vi "VIH Project - Container - Item Rules.vi"(6 "cmd (get)":T9(ring), 8 "error in":errorcluster, 9 "Item Rule":T1, 10 "Item Idx (-1)":i32=-1, 11 "Item Path":path) -> (0 "error out":errorcluster, 1 "Item Rule out":T1, 2 "Item Idx out":i32, 3 "Item Path out":path, 5 "Item Paths":path[](array[path]))   [LabVIEW 2014]
doc: "::: VI Helpeks :::\nCopyright (c) 2000-2026 Konstantin Shifershteyn. All rights reserved."
uses:
  _VIH HelpGen.llb/VIH HelpGen Typedef - Cluster - File Rule.ctl
  _VIH HelpGen.llb/VIH HelpGen Typedef - Enum - Default,Enable,Disable.ctl
  _VIH HelpGen.llb/VIH HelpGen Typedef - Cluster - File Rule - Source Paths.ctl
  _VIH HelpGen.llb/VIH HelpGen Typedef - Cluster - File Rule - Target Paths.ctl
  _VIH HelpGen.llb/VIH HelpGen Typedef - Enum - Description Mode.ctl
  _VIH HelpGen.llb/VIH HelpGen Typedef - Cluster - Control Rule.ctl
  _VIH HelpGen.llb/VIH HelpGen Typedef - Cluster - Enum Value Info.ctl
  _VIH HelpGen.llb/VIH HelpGen Typedef - Cluster - Group Rule - Flags.ctl
panel:
  # "VI Helpeks\nCopyright (c) 2012-2026 Konstantin Shifershteyn"
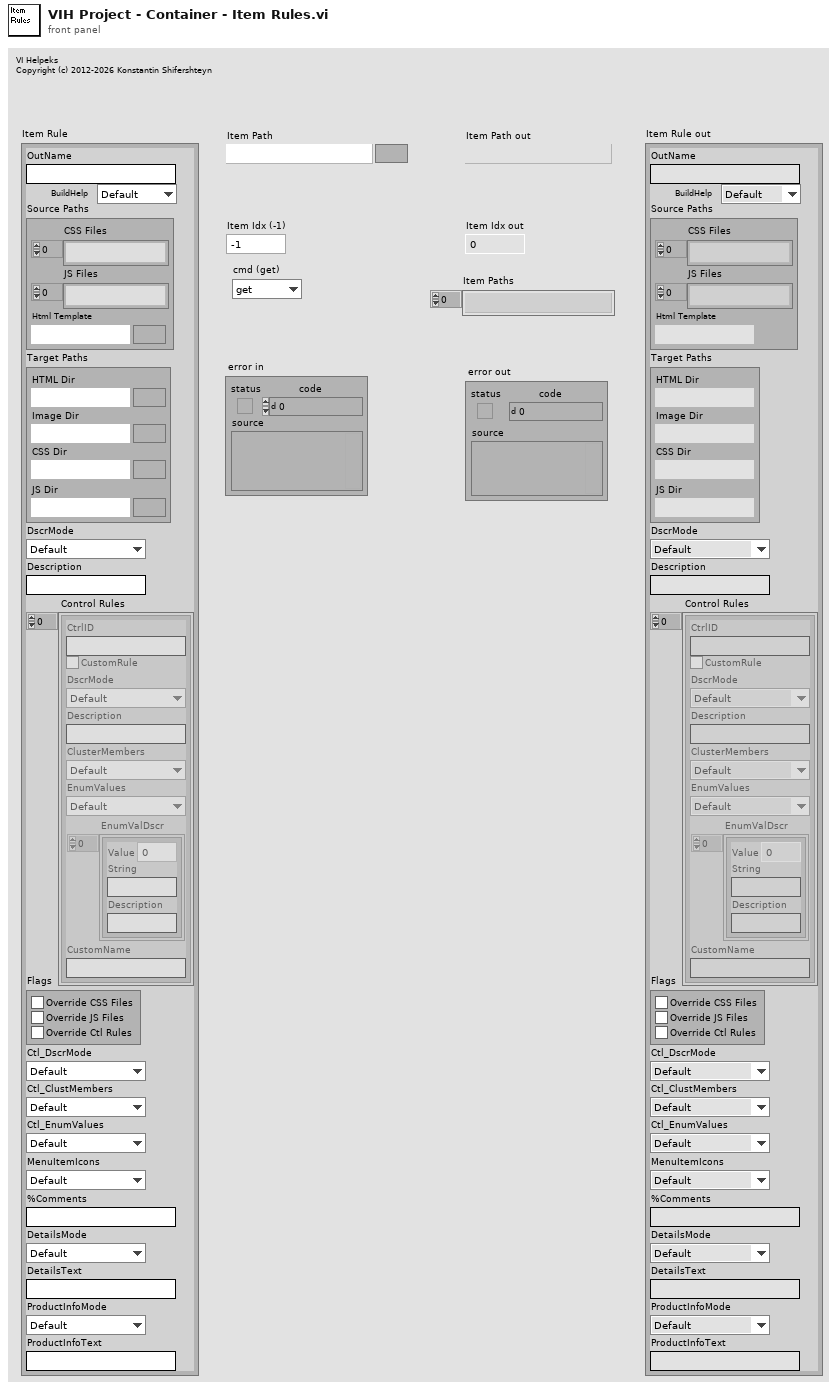
[diagram p1: front panel]
types:
  T1 = typedef "VIH HelpGen Typedef - Cluster - File Rule.ctl" = cluster{"OutName":string, "BuildHelp":T2, "Source Paths":T3, "Target Paths":T4, "DscrMode":T5, "Description":string, "Control Rules":T6[], "Flags":T8, "Ctl_DscrMode":T5, "Ctl_ClustMembers":T2, "Ctl_EnumValues":T2, "MenuItemIcons":T2, "%Comments":string, "DetailsMode":T5, "DetailsText":string, "ProductInfoMode":T2, "ProductInfoText":string}
  T2 = typedef "VIH HelpGen Typedef - Enum - Default,Enable,Disable.ctl" = enum16{"Default", "Enable", "Disable"}
  T3 = typedef "VIH HelpGen Typedef - Cluster - File Rule - Source Paths.ctl" = cluster{"CSS Files":path[], "JS Files":path[], "Html Template":path}
  T4 = typedef "VIH HelpGen Typedef - Cluster - File Rule - Target Paths.ctl" = cluster{"HTML Dir":path, "Image Dir":path, "CSS Dir":path, "JS Dir":path}
  T5 = typedef "VIH HelpGen Typedef - Enum - Description Mode.ctl" = enum16{"Default", "Description", "Description1", "Description2", "Custom", "None"}
  T6 = typedef "VIH HelpGen Typedef - Cluster - Control Rule.ctl" = cluster{"CtrlID":string, "CustomRule":bool, "DscrMode":T5, "Description":string, "ClusterMembers":T2, "EnumValues":T2, "EnumValDscr":T7[], "CustomName":string}
  T7 = typedef "VIH HelpGen Typedef - Cluster - Enum Value Info.ctl" = cluster{"Value":ext, "String":string, "Description":string}
  T8 = typedef "VIH HelpGen Typedef - Cluster - Group Rule - Flags.ctl" = cluster{"Override CSS Files":bool, "Override JS Files":bool, "Override Ctl Rules":bool}
  T9 = enum16{"get", "get all", "set", "Init", "delete", "rename"}
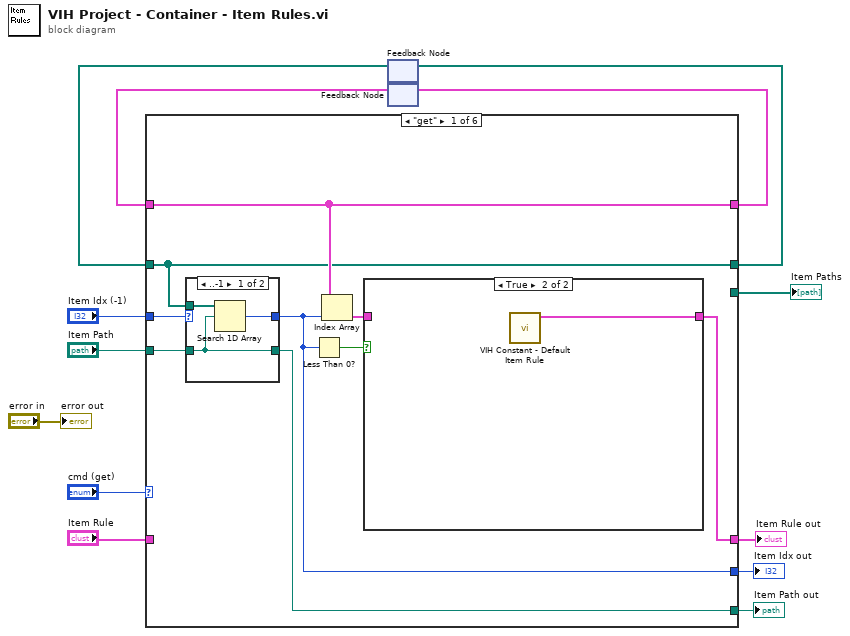
[diagram p0: block diagram]
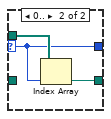
[diagram p3: hidden frame]
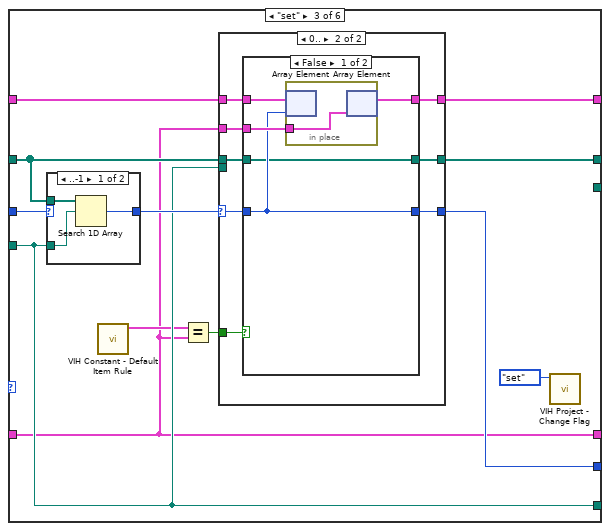
[diagram p5: hidden frame]
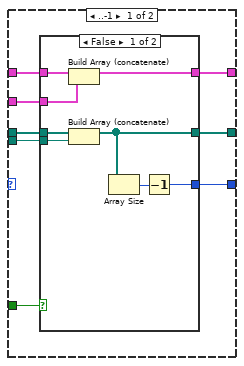
[diagram p7: hidden frame]
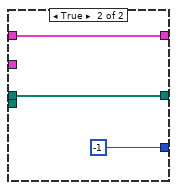
[diagram p8: hidden frame]
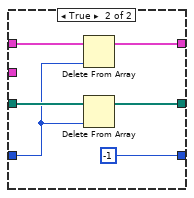
[diagram p9: hidden frame]
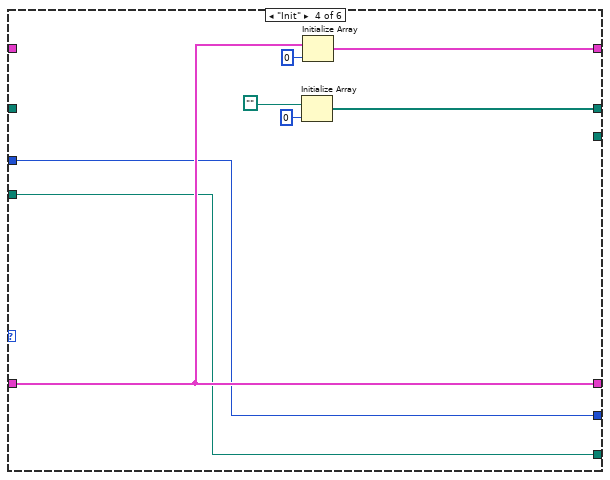
[diagram p10: hidden frame]
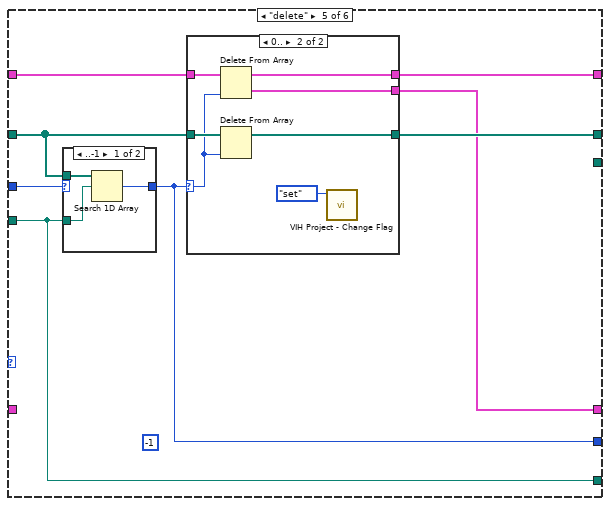
[diagram p11: hidden frame]
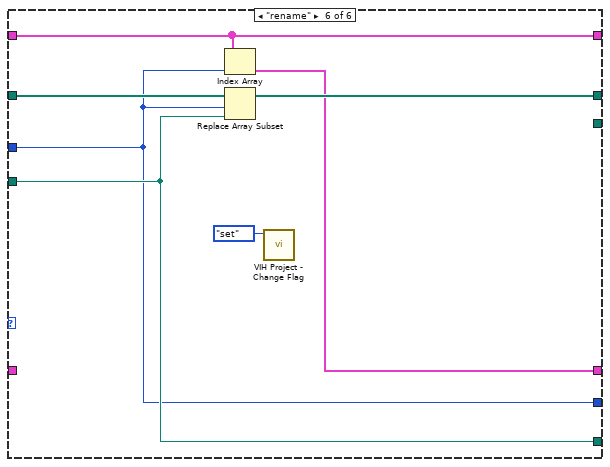
[diagram p14: hidden frame]
diagram:
  n1 = feedback #1() -> (w7:path[])  [unwired: 1 in]
  n2 = feedback #2() -> (w10:T1[])  [unwired: 1 in]
  n3 = case shown="\"get\"" "cmd (get)" {
    tunnel: "Item Rule" -> [_ w33 w37 w93 _ _]
    tunnel: [w22 w35 w46 w97 w105 w122] -> w11
    tunnel: w10 -> [w22 w35 w47 _ w106 w122]
    tunnel: [w20 w34 w45 w94 w104 w125] -> w9
    tunnel: w7 -> [w20 w34 w43 _ w101 w126]
    tunnel: [_ w34 _ _ _ _] -> w8
    tunnel: [w14 w33 w37 w93 w103 w121] -> w6
    tunnel: "Item Idx (-1)" -> [w21 w32 w44 w92 w102 w123]
    tunnel: "Item Path" -> [w19 w31 w40 w91 w100 w124]
    tunnel: [w15 w32 w41 w92 w99 w123] -> w3
    tunnel: [w18 w31 w40 w91 w100 w124] -> w2
    frame "get" {
      n4 = case shown="..-1" w21 {
        selector: w21 -> [_ w28]
        tunnel: [w27 w28] -> w15
        tunnel: w19 -> [w25 _]
        tunnel: w20 -> [w26 w29]
        tunnel: [w25 w30] -> w18
        frame ..-1 {
          n5 = Search 1D Array(1D array=w26, element=w25) -> (index of element=w27:i32)  [unwired: 1 in]
        }
        frame 0.. {
          n6 = Index Array(array=w29, index=w28) -> (element=w30:path)
        }
      }
      n7 = Less Than 0?(x=w15) -> (x < 0?=w17:bool)
      n8 = Index Array(array=w22, index=w15) -> (element=w16:T1)
      n9 = case shown="True" w17 {
        tunnel: [w23 w24] -> w14
        tunnel: w16 -> [w23 _]
        frame False {
        }
        frame True {
          n10 = call "VIH Constant - Default Item Rule.vi"() -> ("Default Item Rule"=w24:T1)  [unwired: 11 in]
        }
      }
    }
    frame "get all" {
    }
    frame "set" {
      n11 = case shown="..-1" w44 {
        selector: w44 -> [_ w51]
        tunnel: [w50 w51] -> w42
        tunnel: w40 -> [w48 _]
        tunnel: w43 -> [w49 _]
        frame ..-1 {
          n12 = Search 1D Array(1D array=w49, element=w48) -> (index of element=w50:i32)  [unwired: 1 in]
        }
        frame 0.. {
        }
      }
      n13 = call "VIH Constant - Default Item Rule.vi"() -> ("Default Item Rule"=w38:T1)  [unwired: 11 in]
      n14 = Equal?(x=w38, y=w37) -> (x = y?=w36:bool)
      n15 = case shown="0.." w42 {
        selector: w42 -> [_ w75]
        tunnel: w47 -> [w59 w78]
        tunnel: [w58 w77] -> w46
        tunnel: w43 -> [w57 w71]
        tunnel: [w53 w72] -> w45
        tunnel: w37 -> [w56 w76]
        tunnel: [w54 w73] -> w41
        tunnel: w40 -> [w55 _]
        tunnel: w36 -> [w52 w74]
        frame ..-1 {
          n16 = case shown="False" w52 {
            tunnel: w59 -> [w67 w70]
            tunnel: [w66 w70] -> w58
            tunnel: w57 -> [w65 w69]
            tunnel: w56 -> [w64 _]
            tunnel: w55 -> [w63 _]
            tunnel: [w61 -1] -> w54
            tunnel: [w60 w69] -> w53
            frame False {
              n17 = Build Array (concatenate)(w67, w64) -> (w66:T1[])
              n18 = Build Array (concatenate)(w65, w63) -> (w60:path[])
              n19 = Array Size(array=w60) -> (size(s)=w62:i32)
              n20 = Decrement(x=w62) -> (x-1=w61:i32)
            }
            frame True {
            }
          }
        }
        frame 0.. {
          n21 = case shown="False" w74 {
            tunnel: w78 -> [w83 w90]
            tunnel: [w82 w89] -> w77
            tunnel: w76 -> [w81 _]
            tunnel: w75 -> [w80 w86]
            tunnel: [w80 -1 ("Item Idx (-1)")] -> w73
            tunnel: [w79 w87] -> w72
            tunnel: w71 -> [w79 w88]
            frame False {
              n22 = in-place {
                in-place-border: w81 -> [w84]
                n23 = in-place-array #3(w83, w80) -> ()  [unwired: 1 out]
                n24 = in-place-array #3(w84) -> (w82:T1[])  [unwired: 1 out]
              }
            }
            frame True {
              n25 = Delete From Array(array=w90, index=w86) -> (array with subset deleted=w89:T1[])  [unwired: 1 in, 1 out]
              n26 = Delete From Array(array=w88, index=w86) -> (array with subset deleted=w87:path[])  [unwired: 1 in, 1 out]
            }
          }
        }
      }
      n27 = call "VIH Project - Change Flag.vi"("cmd (get)"=enum16{"get", "set", "reset"}."set") -> ()  [unwired: 9 in, 2 out]
    }
    frame "Init" {
      n28 = Initialize Array(path "", 0 ("dimension size")) -> (w94:path[])
      n29 = Initialize Array(w93, 0 ("dimension size")) -> (w97:T1[])
    }
    frame "delete" {
      (unwired) -1 ("Item Idx (-1)")
      n30 = case shown="..-1" w102 {
        selector: w102 -> [_ w110]
        tunnel: [w109 w110] -> w99
        tunnel: w100 -> [w107 _]
        tunnel: w101 -> [w108 _]
        frame ..-1 {
          n31 = Search 1D Array(1D array=w108, element=w107) -> (index of element=w109:i32)  [unwired: 1 in]
        }
        frame 0.. {
        }
      }
      n32 = case shown="0.." w99 {
        selector: w99 -> [_ w114]
        tunnel: w106 -> [w112 w119]
        tunnel: [w112 w118] -> w105
        tunnel: w101 -> [w111 w117]
        tunnel: [w111 w116] -> w104
        tunnel: [_ w115] -> w103
        frame ..-1 {
        }
        frame 0.. {
          n33 = Delete From Array(array=w119, index=w114) -> (deleted portion=w115:T1, array with subset deleted=w118:T1[])  [unwired: 1 in]
          n34 = Delete From Array(array=w117, index=w114) -> (array with subset deleted=w116:path[])  [unwired: 1 in, 1 out]
          n35 = call "VIH Project - Change Flag.vi"("cmd (get)"=enum16{"get", "set", "reset"}."set") -> ()  [unwired: 9 in, 2 out]
        }
      }
    }
    frame "rename" {
      n36 = Index Array(array=w122, index=w123) -> (element=w121:T1)
      n37 = Replace Array Subset(array=w126, new element=w124, index=w123) -> (w125:path[])
      n38 = call "VIH Project - Change Flag.vi"("cmd (get)"=enum16{"get", "set", "reset"}."set") -> ()  [unwired: 9 in, 2 out]
    }
  }
  "Item Path out" <- w2
  "Item Rule out" <- w6
  "Item Paths" <- w8
  "Item Idx out" <- w3
  n39 = feedback-in #1(w9) -> ()
  n40 = feedback-in #2(w11) -> ()
  "error out" <- "error in"
